vi "getConnectionPoint.vi"(0 "reference":refnum<class "CallNode.lvclass">, 1 "direction":refnum<class "Direction.lvclass">, 5 "error in (no error)":errorcluster) -> (14 "reference out":refnum<class "CallNode.lvclass">, 15 "point2D":T1 {"y" format="%.2f"; "x" format="%.2f"}, 19 "error out":errorcluster)   [LabVIEW 2020, in "CallNode.lvclass"]
uses:
  <resource>/Framework/Providers/Open_GDS/UML/CallNode_class/CallNode.lvclass
  C:/Program Files (x86)/National Instruments/LabVIEW 2020/resource/Framework/Providers/Open_GDS/UML/RectangularNode_class/RectangularNode.lvclass
  <resource>/Framework/Providers/Open_GDS/UML/Direction_class/Direction.lvclass
  <resource>/Framework/Providers/Open_GDS/UML/General/Point/Point Point2D.ctl
  <resource>/Framework/Providers/Open_GDS/UML/RectangularNode_class/RectangularNode.lvclass
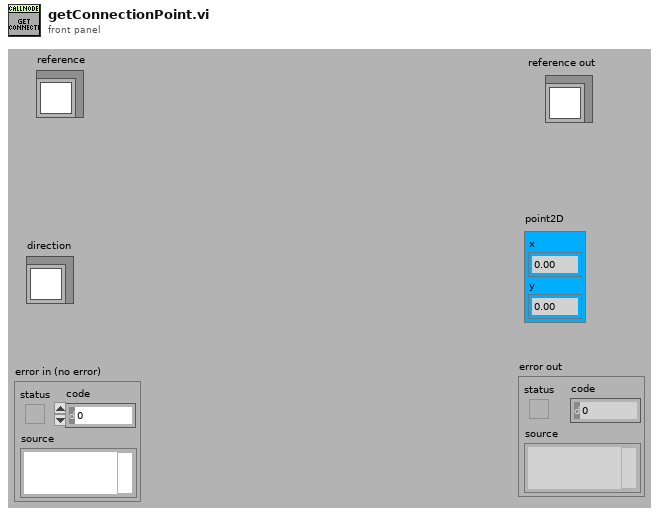
[diagram p1: front panel]
types:
  T1 = typedef "Point Point2D.ctl" = cluster{"x":dbl, "y":dbl}
  T2 = typedef "RectangularNode.lvclass/ObjectAttributes.ctl" = cluster{"bounds":T3}
  T3 = typedef "Rectangle Rectangle2D.ctl" = cluster{"x":dbl, "y":dbl, "width":dbl, "height":dbl}
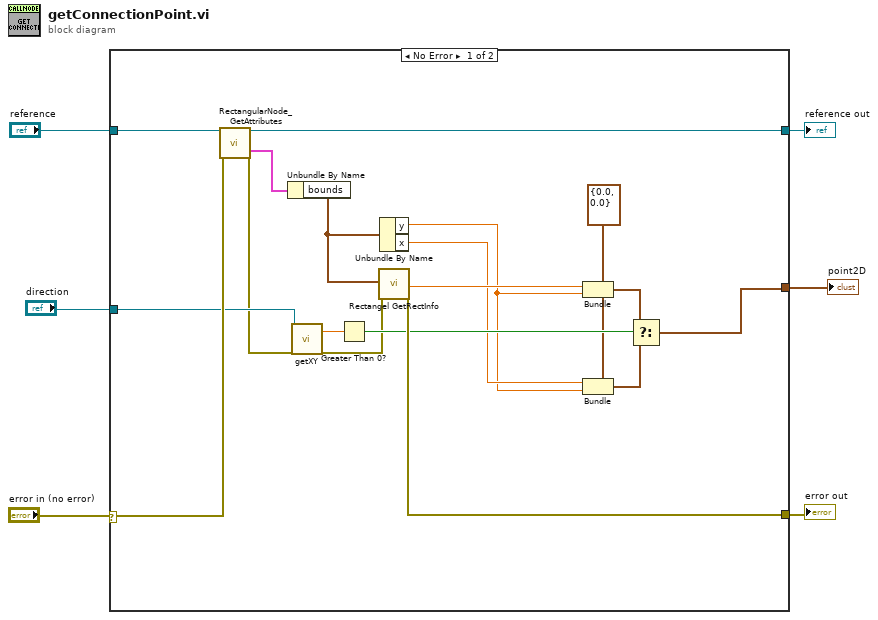
[diagram p0: block diagram]
diagram:
  n1 = case shown="No Error" "error in (no error)" {
    selector: "error in (no error)" -> [w21 w25]
    tunnel: "reference" -> [w24 w26]
    tunnel: [w23 w25] -> w5
    tunnel: [w22 w26] -> w4
    tunnel: "direction" -> [w20 _]
    tunnel: [w19 _] -> w1
    frame No Error {
      w16 = T1 {"x"=0.0, "y"=0.0} ("point2D")
      n2 = call <resource>:"RectangularNode_GetAttributes.vi"("reference in"=w24, "error in (no error)"=w21) -> ("reference out"=w22:refnum<class "CallNode.lvclass">, "Data"=w7:T2, "error out"=w9:errorcluster)  [unwired: 14 in, 1 out]
      n3 = Unbundle By Name(w7) -> ("bounds"=w13:T3)
      n4 = call <resource>:"getXY.vi"("reference"=w20, "error in (no error)"=w9) -> ("x"=w18:dbl, "error out"=w10:errorcluster)  [unwired: 16 out]
      n5 = Greater Than 0?(x=w18) -> (x > 0?=w17:bool)
      n6 = call <resource>:"Rectangel GetRectInfo.vi"("bounds"=w13, "error in (no error)"=w10) -> ("maxX"=w14:dbl, "error out"=w23:errorcluster)  [unwired: 16 out]
      n7 = Unbundle By Name(w13) -> ("y"=w8:dbl, "x"=w11:dbl)
      n8 = Bundle(cluster=w16, "x"=w14, "y"=w8) -> (w15:T1)
      n9 = Bundle(cluster=w16, "x"=w11, "y"=w8) -> (w12:T1)
      n10 = Select(t=w15, s=w17, f=w12) -> (s? t:f=w19:T1)
    }
    frame Error {
    }
  }
  "reference out" <- w4
  "error out" <- w5
  "point2D" <- w1
